vi "Power Meter.vi"(8 "error in (no error)":errorcluster, 10 "Gain":dbl=1.02, 11 "True Power (W)":dbl) -> (0 "error out":errorcluster, 3 "Reading (W)":dbl format="%#_3g")   [LabVIEW 2026]
panel:
  in  "Offset (W)":dbl=0.005
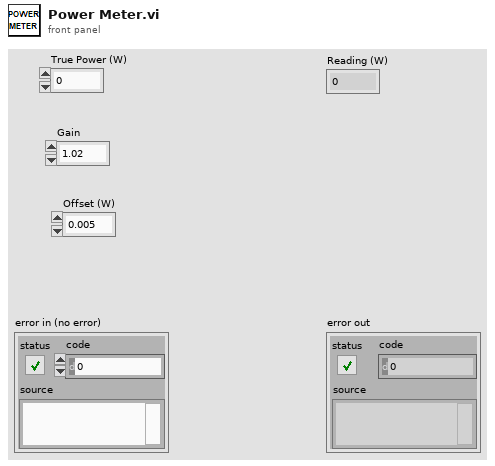
[diagram p1: front panel]
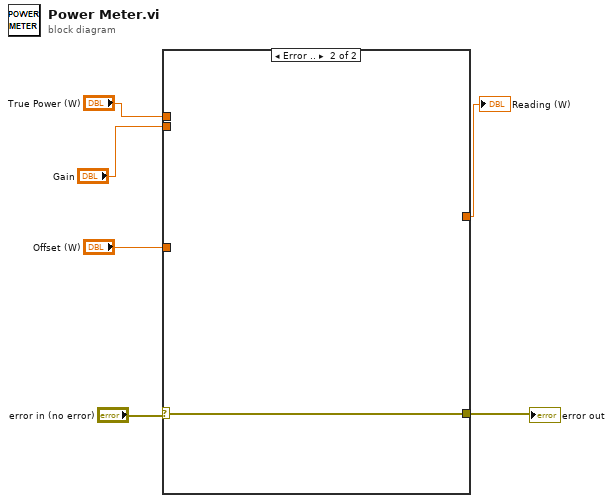
[diagram p0: block diagram]
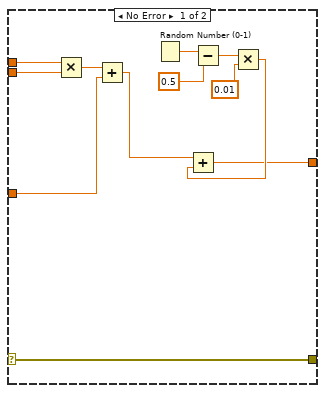
[diagram p2: hidden frame]
diagram:
  n1 = case shown="Error .." "error in (no error)" {
    selector: "error in (no error)" -> [w18 w19]
    tunnel: [w18 w19] -> w5
    tunnel: "True Power (W)" -> [w17 _]
    tunnel: "Gain" -> [w16 _]
    tunnel: "Offset (W)" -> [w14 _]
    tunnel: [w7 _] -> w1
    frame No Error {
      n2 = Multiply(x=w17, y=w16) -> (x*y=w15:dbl)
      n3 = Add(x=w15, y=w14) -> (x+y=w9:dbl)
      n4 = Random Number (0-1)() -> (number: 0 to 1=w13:dbl)
      n5 = Subtract(x=w13, y=0.5) -> (x-y=w11:dbl)
      n6 = Multiply(x=w11, y=0.01) -> (x*y=w8:dbl)
      n7 = Add(x=w9, y=w8) -> (x+y=w7:dbl)
    }
    frame Error {
    }
  }
  "Reading (W)" <- w1
  "error out" <- w5
